vi "Mode#.vi"(11 "MR all data":bool[](array[boolean])) -> (3 "Mode#":i32)   [LabVIEW 2018]
panel:
  out "x < y?":bool
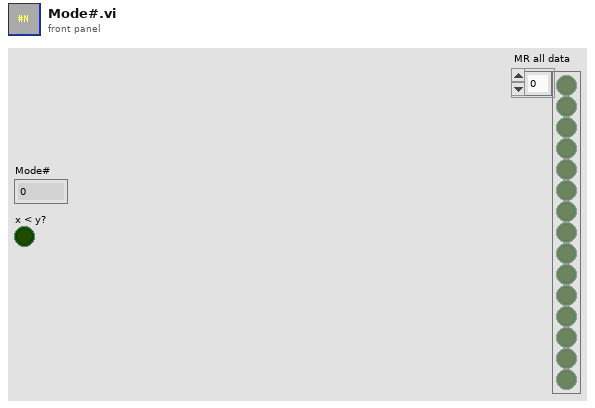
[diagram p1: front panel]
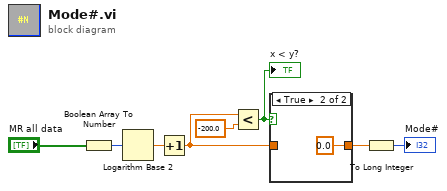
[diagram p0: block diagram]
diagram:
  n1 = Boolean Array To Number(Boolean array="MR all data") -> (number=w2:u32)
  n2 = Logarithm Base 2(1:w2) -> (0:w3:dbl)
  n3 = Increment(x=w3) -> (x+1=w6:dbl)
  n4 = Less?(x=w6, y=-200.0) -> (x < y?=w4:bool)
  "x < y?" <- w4
  n5 = case shown="True" w4 {
    tunnel: w6 -> [w9 _]
    tunnel: [w9 0.0] -> w8
    frame False {
    }
    frame True {
    }
  }
  n6 = To Long Integer(number=w8) -> (32bit integer=→"Mode#":i32)
